vi "Native_SetNumericRepresentation.vi"() -> ()   [LabVIEW 2024]
panel:
  out "error out":errorcluster caption="错误输出"
  in  "representation":u32=3
  in  "numeric_id":u32
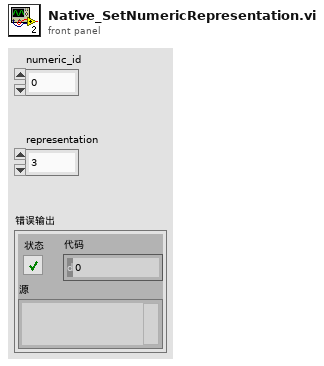
[diagram p1: front panel]
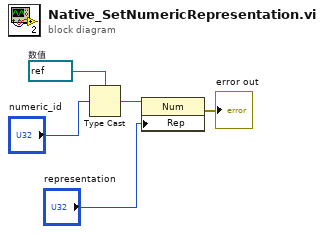
[diagram p0: block diagram]
diagram:
  w4 = refnum<vi> refnum  # 数值
  n1 = Type Cast ("强制类型转换")(type=w4, x="numeric_id") -> (*(type *) &x=w3:refnum<vi>)
  n2 = property on="属性节点" class="Num"(reference=w3, "Rep"="representation") -> (error out=→"error out":errorcluster)  [unwired: 1 in, 1 out]
